vi "test non object message.vi"(8 "error in (no error)":errorcluster) -> (0 "error out":errorcluster, 3 "body":string)   [LabVIEW 2020, in "MCP Server tests.lvlib"]
doc: "A body that is valid JSON but neither an object nor an array (a number, a string, true, false, null) is an invalid request: JSON-RPC error -32600 with id null, not a parse error."
uses:
  MCP Server tests.lvlib
  <vilib>/JDP Science/JSONtext/Next JSON Value.vi
  <vilib>/JDP Science/JSONtext/String Subset.vi
  <vilib>/JDP Science/JSONtext/Parsing/Advance past next JSON Value (inlined COPY).vi
  <vilib>/JDP Science/JSONtext/Parsing/Advance past whitespace.vi
  <vilib>/JDP Science/JSONtext/Parsing/Advance past String.vi
  <vilib>/JDP Science/JSONtext/Parsing/Advance past Number.vi
  <vilib>/JDP Science/JSONtext/Parsing/Advance past Line Ending.vi
  <vilib>/JDP Science/JSONtext/Parsing/Parse Full Path or Item Name.vi
  <vilib>/JDP Science/JSONtext/Parsing/Advance past Array.vi
  <vilib>/JDP Science/JSONtext/Parsing/Advance past Object.vi
  <vilib>/JDP Science/JSONtext/support/Error Cluster From Code.vi
  <vilib>/JDP Science/JSONtext/Offset/Find Item Locations by Path.vi
  <vilib>/addons/_JKI Toolkits/Caraya/classes/Test/Test.lvclass
  <vilib>/JDP Science/JSONtext/JSONtext.lvlib
  <vilib>/addons/_JKI Toolkits/Caraya/classes/Assert/Assert.lvclass
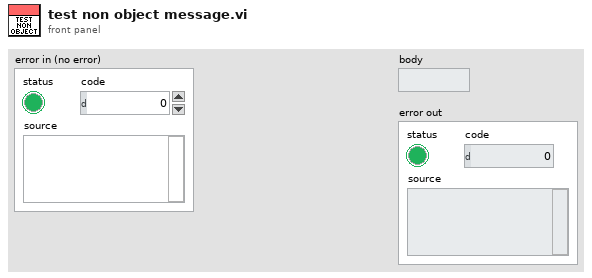
[diagram p1: front panel]
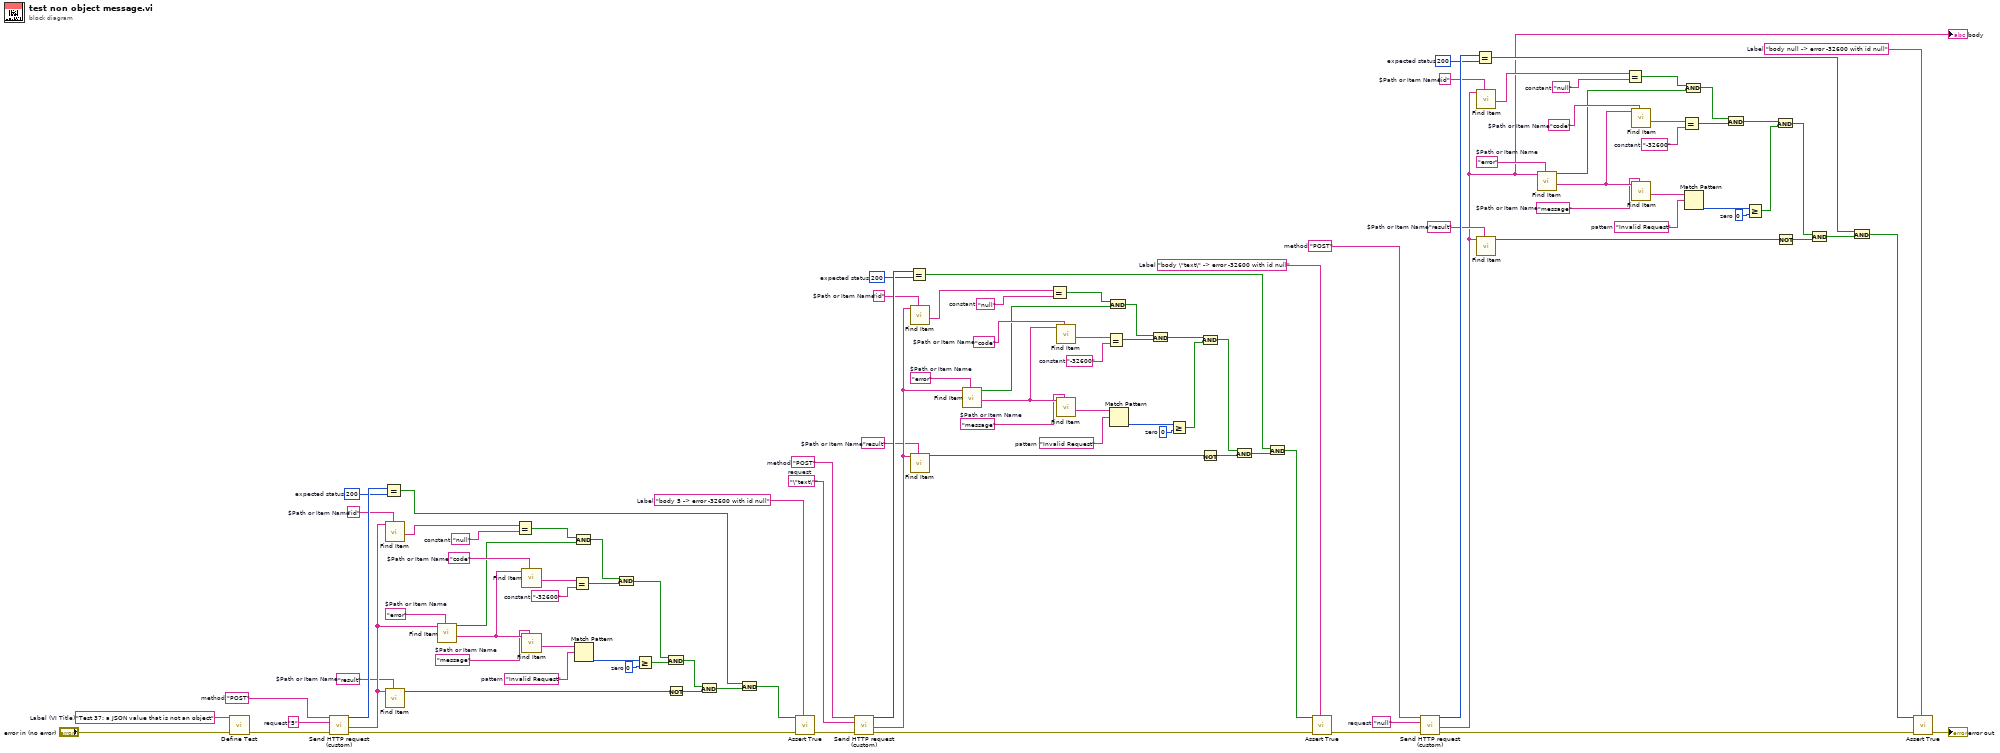
[diagram p0: block diagram]
diagram:
  w3 = "body null -> error -32600 with id null"  # Label
  w17 = 0  # zero
  w19 = "Invalid Request"  # pattern
  w21 = "-32600"  # constant
  w23 = "null"  # constant
  w25 = "result"  # $Path or Item Name
  w26 = "message"  # $Path or Item Name
  w28 = "code"  # $Path or Item Name
  w29 = "error"  # $Path or Item Name
  w30 = "id"  # $Path or Item Name
  w31 = 200  # expected status
  w34 = "null"  # request
  w35 = "POST"  # method
  w36 = "body \"text\" -> error -32600 with id null"  # Label
  w50 = 0  # zero
  w52 = "Invalid Request"  # pattern
  w54 = "-32600"  # constant
  w56 = "null"  # constant
  w58 = "result"  # $Path or Item Name
  w60 = "message"  # $Path or Item Name
  w62 = "code"  # $Path or Item Name
  w63 = "error"  # $Path or Item Name
  w64 = "id"  # $Path or Item Name
  w65 = 200  # expected status
  w68 = "\"text\""  # request
  w69 = "POST"  # method
  w70 = "body 5 -> error -32600 with id null"  # Label
  w84 = 0  # zero
  w86 = "Invalid Request"  # pattern
  w88 = "-32600"  # constant
  w90 = "null"  # constant
  w92 = "result"  # $Path or Item Name
  w94 = "message"  # $Path or Item Name
  w96 = "code"  # $Path or Item Name
  w97 = "error"  # $Path or Item Name
  w98 = "id"  # $Path or Item Name
  w99 = 200  # expected status
  w102 = "5"  # request
  w103 = "POST"  # method
  w105 = "Test 37: a JSON value that is not an object"  # Label (VI Title)
  n1 = call <vilib>:"Define Test.vi"("error in (no error)"="error in (no error)", "Label (VI Title)"=w105) -> ("error out"=w101:errorcluster)  [unwired: 8 in, 1 out]
  n2 = call "Send HTTP request (custom).vi"("error in (no error)"=w101, "request"=w102, "method"=w103) -> ("error out"=w71:errorcluster, "response"=w93:string, "status code"=w100:i32)  [unwired: 5 in, 1 out]
  n3 = Equal?(x=w100, y=w99) -> (x = y?=w74:bool)
  n4 = call <vilib>:"Find Item.vi"("$Path or Item Name"=w98, "JSON"=w93) -> ("<JSON>"=w91:string)  [unwired: 6 in, 3 out]
  n5 = call <vilib>:"Find Item.vi"("$Path or Item Name"=w92, "JSON"=w93) -> ("Found"=w83:bool)  [unwired: 6 in, 3 out]
  n6 = call <vilib>:"Find Item.vi"("$Path or Item Name"=w97, "JSON"=w93) -> ("<JSON>"=w95:string, "Found"=w81:bool)  [unwired: 6 in, 2 out]
  n7 = Equal?(x=w91, y=w90) -> (x = y?=w82:bool)
  n8 = call <vilib>:"Find Item.vi"("$Path or Item Name"=w96, "JSON"=w95) -> ("<JSON>"=w89:string)  [unwired: 6 in, 3 out]
  n9 = call <vilib>:"Find Item.vi"("$Path or Item Name"=w94, "JSON"=w95) -> ("<JSON>"=w87:string)  [unwired: 6 in, 3 out]
  n10 = Equal?(x=w89, y=w88) -> (x = y?=w79:bool)
  n11 = And(x=w82, y=w81) -> (x .and. y?=w80:bool)
  n12 = Match Pattern(string=w87, regular expression=w86) -> (offset past match=w85:i32)  [unwired: 1 in, 3 out]
  n13 = And(x=w80, y=w79) -> (x .and. y?=w78:bool)
  n14 = Greater Or Equal?(x=w85, y=w84) -> (x >= y?=w77:bool)
  n15 = And(x=w78, y=w77) -> (x .and. y?=w76:bool)
  n16 = Not(x=w83) -> (.not. x?=w75:bool)
  n17 = And(x=w76, y=w75) -> (x .and. y?=w73:bool)
  n18 = And(x=w74, y=w73) -> (x .and. y?=w72:bool)
  n19 = call <vilib>:"Assert True.vi"("Label"=w70, "error in (no error)"=w71, "True?"=w72) -> ("error out"=w67:errorcluster)  [unwired: 7 in, 1 out]
  n20 = call "Send HTTP request (custom).vi"("error in (no error)"=w67, "request"=w68, "method"=w69) -> ("error out"=w37:errorcluster, "response"=w59:string, "status code"=w66:i32)  [unwired: 5 in, 1 out]
  n21 = Equal?(x=w66, y=w65) -> (x = y?=w40:bool)
  n22 = call <vilib>:"Find Item.vi"("$Path or Item Name"=w64, "JSON"=w59) -> ("<JSON>"=w57:string)  [unwired: 6 in, 3 out]
  n23 = call <vilib>:"Find Item.vi"("$Path or Item Name"=w58, "JSON"=w59) -> ("Found"=w49:bool)  [unwired: 6 in, 3 out]
  n24 = call <vilib>:"Find Item.vi"("$Path or Item Name"=w63, "JSON"=w59) -> ("<JSON>"=w61:string, "Found"=w47:bool)  [unwired: 6 in, 2 out]
  n25 = Equal?(x=w57, y=w56) -> (x = y?=w48:bool)
  n26 = call <vilib>:"Find Item.vi"("$Path or Item Name"=w62, "JSON"=w61) -> ("<JSON>"=w55:string)  [unwired: 6 in, 3 out]
  n27 = call <vilib>:"Find Item.vi"("$Path or Item Name"=w60, "JSON"=w61) -> ("<JSON>"=w53:string)  [unwired: 6 in, 3 out]
  n28 = Equal?(x=w55, y=w54) -> (x = y?=w45:bool)
  n29 = And(x=w48, y=w47) -> (x .and. y?=w46:bool)
  n30 = Match Pattern(string=w53, regular expression=w52) -> (offset past match=w51:i32)  [unwired: 1 in, 3 out]
  n31 = And(x=w46, y=w45) -> (x .and. y?=w44:bool)
  n32 = Greater Or Equal?(x=w51, y=w50) -> (x >= y?=w43:bool)
  n33 = And(x=w44, y=w43) -> (x .and. y?=w42:bool)
  n34 = Not(x=w49) -> (.not. x?=w41:bool)
  n35 = And(x=w42, y=w41) -> (x .and. y?=w39:bool)
  n36 = And(x=w40, y=w39) -> (x .and. y?=w38:bool)
  n37 = call <vilib>:"Assert True.vi"("Label"=w36, "error in (no error)"=w37, "True?"=w38) -> ("error out"=w33:errorcluster)  [unwired: 7 in, 1 out]
  n38 = call "Send HTTP request (custom).vi"("error in (no error)"=w33, "request"=w34, "method"=w35) -> ("error out"=w4:errorcluster, "response"=w2:string, "status code"=w32:i32)  [unwired: 5 in, 1 out]
  "body" <- w2
  n39 = Equal?(x=w32, y=w31) -> (x = y?=w7:bool)
  n40 = call <vilib>:"Find Item.vi"("$Path or Item Name"=w30, "JSON"=w2) -> ("<JSON>"=w24:string)  [unwired: 6 in, 3 out]
  n41 = call <vilib>:"Find Item.vi"("$Path or Item Name"=w25, "JSON"=w2) -> ("Found"=w16:bool)  [unwired: 6 in, 3 out]
  n42 = call <vilib>:"Find Item.vi"("$Path or Item Name"=w29, "JSON"=w2) -> ("<JSON>"=w27:string, "Found"=w14:bool)  [unwired: 6 in, 2 out]
  n43 = Equal?(x=w24, y=w23) -> (x = y?=w15:bool)
  n44 = call <vilib>:"Find Item.vi"("$Path or Item Name"=w28, "JSON"=w27) -> ("<JSON>"=w22:string)  [unwired: 6 in, 3 out]
  n45 = call <vilib>:"Find Item.vi"("$Path or Item Name"=w26, "JSON"=w27) -> ("<JSON>"=w20:string)  [unwired: 6 in, 3 out]
  n46 = Equal?(x=w22, y=w21) -> (x = y?=w12:bool)
  n47 = And(x=w15, y=w14) -> (x .and. y?=w13:bool)
  n48 = Match Pattern(string=w20, regular expression=w19) -> (offset past match=w18:i32)  [unwired: 1 in, 3 out]
  n49 = And(x=w13, y=w12) -> (x .and. y?=w11:bool)
  n50 = Greater Or Equal?(x=w18, y=w17) -> (x >= y?=w10:bool)
  n51 = And(x=w11, y=w10) -> (x .and. y?=w9:bool)
  n52 = Not(x=w16) -> (.not. x?=w8:bool)
  n53 = And(x=w9, y=w8) -> (x .and. y?=w6:bool)
  n54 = And(x=w7, y=w6) -> (x .and. y?=w5:bool)
  n55 = call <vilib>:"Assert True.vi"("Label"=w3, "error in (no error)"=w4, "True?"=w5) -> ("error out"=→"error out":errorcluster)  [unwired: 7 in, 1 out]
